vi "Get Subscriber Count.vi"(8 "error in (no error)":errorcluster, 11 "Publisher Reference":T1 {"refnum" format="%.0x"}) -> (0 "error out":errorcluster, 1 "Best Effort":u32, 2 "Backpressure":u32)   [LabVIEW 2021, in "Iceoryx.lvlib"]
doc: "Returns the number of subscribers currently attached to the backpressure and best effort queues."
uses:
  Iceoryx.lvlib
  SubVIs/Convert Error Core.vi
  Refnum/Typedef/Raw Publisher Refnum.ctl
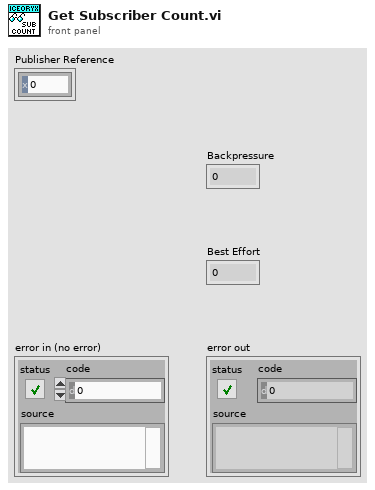
[diagram p1: front panel]
types:
  T1 = typedef "Iceoryx.lvlib/Raw Publisher Refnum.ctl" = cluster{"refnum":u64, "Raw Pub":enum8{"rawpub"}}
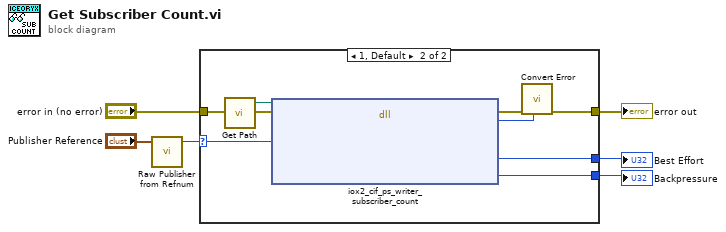
[diagram p0: block diagram]
diagram:
  n1 = call "Raw Publisher from Refnum.vi"("Raw Publisher Refnum"="Publisher Reference") -> ("Raw Publisher U64"=w1:u64)  [unwired: 4 in]
  n2 = case shown="1, Default" w1 {
    selector: w1 -> [_ w12]
    tunnel: "error in (no error)" -> [w7 w9]
    tunnel: [w7 w8] -> w4
    tunnel: [_ w11] -> w3
    tunnel: [_ w10] -> w2
    frame 0 {
    }
    frame 1, Default {
      n3 = call "Get Path.vi"() -> ("libiox2_cif path"=w15:path)  [unwired: 4 in]
      n4 = dll-call lib="D:/dev/iceoryx2_lvwrapper/dist/iox2_cif.dll" fn="iox2_cif_ps_writer_subscriber_count"(path in=w15, error in=w9, "writer"=w12) -> (error out=w14:errorcluster, "return type"=w13:i32, "best_effort"=w11:u32, "backpressure"=w10:u32)  [unwired: 4 in, 1 out]
      n5 = call "Convert Error.vi"("return type"=w13, "error in (no error)"=w14) -> ("error out"=w8:errorcluster)  [unwired: 9 in]
    }
  }
  "error out" <- w4
  "Best Effort" <- w3
  "Backpressure" <- w2
